vi "Set Tag.vi"(8 "error in (no error)":errorcluster, 10 "Tag":string, 11 "CTI_Channel in":refnum<class "CTI_Channel.lvclass">) -> (0 "error out":errorcluster, 3 "CTI_Channel out":refnum<class "CTI_Channel.lvclass">)   [LabVIEW 2021, in "CTI_Channel.lvclass"]
uses:
  CTI_Channel.lvclass
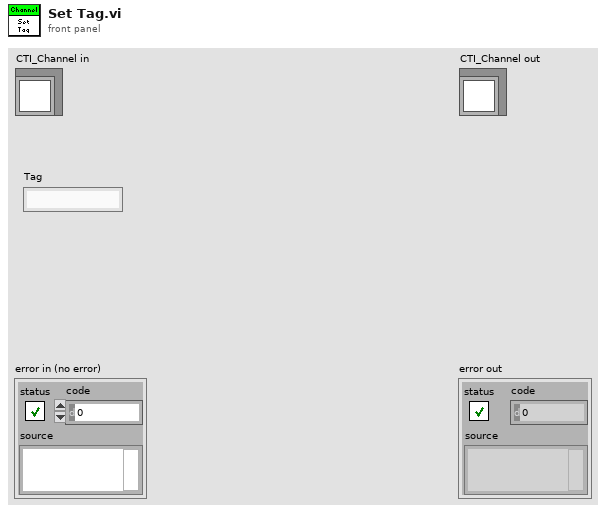
[diagram p1: front panel]
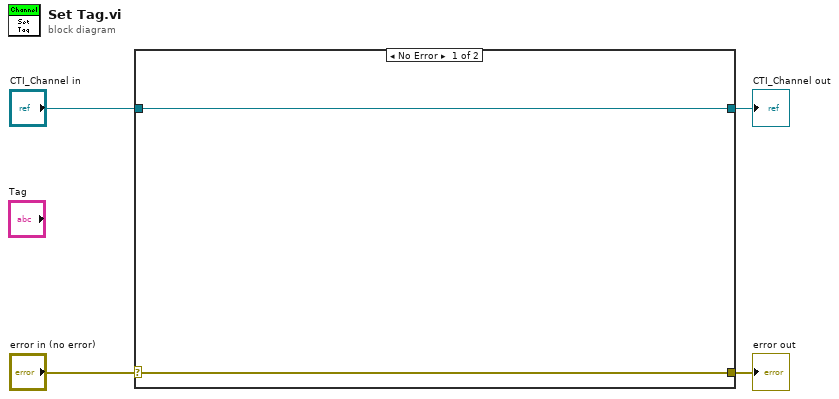
[diagram p0: block diagram]
diagram:
  n1 = case shown="No Error" "error in (no error)" {
    selector: "error in (no error)" -> [w5 w8]
    tunnel: [w5 w8] -> w3
    tunnel: [w6 w7] -> w1
    tunnel: "CTI_Channel in" -> [w6 w7]
    frame No Error {
    }
    frame Error {
    }
  }
  "error out" <- w3
  "CTI_Channel out" <- w1
